vi "UE_Measured_Displacement.vi"(1 "initial_mm":dbl, 2 "final_mm":dbl) -> (0 "delta_mm":dbl)   [LabVIEW 2026]
doc: "INTENT: Compute signed displacement between two valid position samples. INPUTS: final_mm (double), initial_mm (double). OUTPUTS: delta_mm (double). DESIGN CONSTRAINT: REQUIREMENTS: SRS-F-020. No physical hardware side effects. Acceptance requires native LabVIEW compilation and behavioral testing."
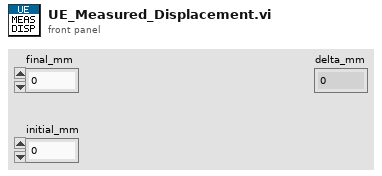
[diagram p1: front panel]
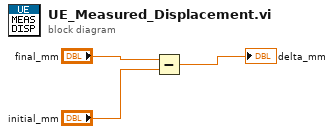
[diagram p0: block diagram]
diagram:
  n1 = Subtract(x="final_mm", y="initial_mm") -> (x-y=→"delta_mm":dbl)
